vi "HostMem GetPointer.vi"(8 "error in (no error)":errorcluster, 11 "HostMem in":refnum<class "HostMem.lvclass">) -> (0 "error out":errorcluster, 2 "PointerData":T1, 3 "HostMem out":refnum<class "HostMem.lvclass">)   [LabVIEW 2020, in "OpenLvVision_OpenCv.lvlib" / "Cuda.lvlib" / "HostMem.lvclass"]
doc: "Returns the raw memory pointer to the pinned data buffer for zero-copy access.\n\nThis increments the OpenCV reference count. To prevent memory leaks, the generated handlePtr must be freed after use, either by the external library via the releaseCallback, or explicitly in LabVIEW using the \"HostMem ReleasePointer\" VI."
uses:
  HostMem.lvclass
  C:/Users/lukas/Documents/OpenLvVision_OpenCv/SourceCode/LabView/OpenLvVision_OpenCv/_LvHelpers/EdvrObject/EdvrObject.lvclass
  TypeDef/HostMem PointerData.ctl
  TypeDef/cvType.ctl
  _LvHelpers/EdvrObject/EdvrObject.lvclass/EdvrObject.ctl
  OpenLvVision_OpenCv.lvlib
  <vilib>/Utility/error.llb/Error Cluster From Error Code.vi
  <vilib>/ErrorRing/Error Ring.xnode
  _LvHelpers/EdvrObject/EdvrObject.lvclass
  Dlls/OlvOpenCvWrapper.dll
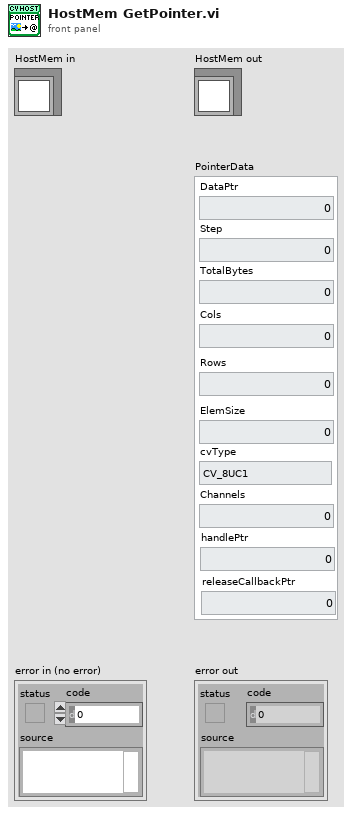
[diagram p1: front panel]
types:
  T1 = typedef "OpenLvVision_OpenCv.lvlib/HostMem PointerData.ctl" = cluster{"DataPtr":u64, "Step":i64, "TotalBytes":u64, "Cols":i32, "Rows":i32, "ElemSize":i32, "cvType":T2, "Channels":i32, "handlePtr":u64, "releaseCallbackPtr":u64}
  T2 = typedef "OpenLvVision_OpenCv.lvlib/cvType.ctl" = enum32{"CV_8UC1", "CV_8SC1", "CV_16UC1", "CV_16SC1", "CV_32SC1", "CV_32FC1", "CV_64FC1", "CV_16FC1", "CV_8UC2", "CV_8SC2", "CV_16UC2", "CV_16SC2", "CV_32SC2", "CV_32FC2", "CV_64FC2", "CV_16FC2", "CV_8UC3", "CV_8SC3", "CV_16UC3", "CV_16SC3", "CV_32SC3", "CV_32FC3", "CV_64FC3", "CV_16FC3", "CV_8UC4", "CV_8SC4", "CV_16UC4", "CV_16SC4", "CV_32SC4", "CV_32FC4", "CV_64FC4", "CV_16FC4"}
  T3 = typedef "OpenLvVision_OpenCv.lvlib/EdvrObject.lvclass/Edvr.ctl" = refnum<data-value>
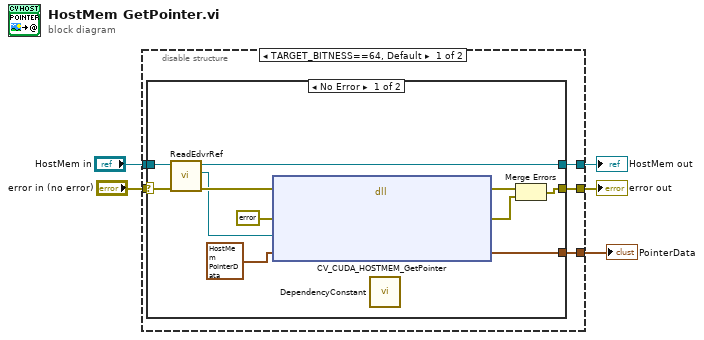
[diagram p0: block diagram]
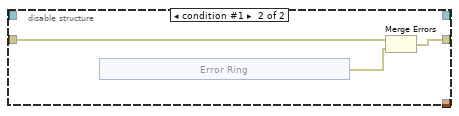
[diagram p3: hidden frame]
diagram:
  n1 = disable-structure shown="TARGET_BITNESS==64, Default" {
    disable-tunnel: "error in (no error)" -> [w10 w25]
    disable-tunnel: [w9 w26] -> w4
    disable-tunnel: "HostMem in" -> [w8 _]
    disable-tunnel: [w7 _] -> w2
    disable-tunnel: [w6 _] -> w1
    frame condition #0 (active) {
      n2 = case shown="No Error" w10 {
        selector: w10 -> [w18 w23]
        tunnel: [w13 w23] -> w9
        tunnel: w8 -> [w17 w22]
        tunnel: [w14 w22] -> w7
        tunnel: [w12 _] -> w6
        frame No Error {
          n3 = call "ReadEdvrRef.vi"("error in (no error)"=w18, "EdvrObject in"=w17) -> ("error out"=w16:errorcluster, "Edvr"=w15:T3, "EdvrObject out"=w14:refnum<class "HostMem.lvclass">)  [unwired: 7 in]
          n4 = dll-call lib="C:/Users/lukas/Documents/OpenLvVision_OpenCv/SourceCode/LabView/OpenLvVision_OpenCv/Dlls/OlvOpenCvWrapper.dll" fn="CV_CUDA_HOSTMEM_GetPointer"(error in=w16, "Error"=errorcluster {"status"=FALSE, "code"=0, "source"=""} ("error out"), "edvrRef"=w15, "Pointer"=T1 {"DataPtr"=0, "Step"=0, "TotalBytes"=0, "Cols"=0, "Rows"=0, "ElemSize"=0, "cvType"=enum."CV_8UC1", "Channels"=0, "handlePtr"=0, "releaseCallbackPtr"=0} ("PointerData")) -> (error out=w21:errorcluster, "Error"=w20:errorcluster, "Pointer"=w12:T1)  [unwired: 4 in, 1 out]
          n5 = call "DependencyConstant.vi"() -> ()  [unwired: 12 in]
          n6 = Merge Errors(w21, w20) -> (w13:errorcluster)
        }
        frame Error {
        }
      }
    }
    frame condition #1 {
      n7 = xnode "Error Ring"() -> ("error out"=w24:errorcluster)
      n8 = Merge Errors(w25, w24) -> (w26:errorcluster)
    }
  }
  "error out" <- w4
  "HostMem out" <- w2
  "PointerData" <- w1
